vi "Username Dialog.vi"(7 "Address":string, 8 "Error In":errorcluster, 11 "Username In":string="cfield") -> (0 "Error Out":errorcluster, 3 "Username Out":string="cfield")   [LabVIEW 2017, in "Tests.lvlib"]
uses:
  Tests.lvlib
  <vilib>/Utility/miscctls.llb/LVSelectionTypeDef.ctl
panel:
  out "Host":string="USERNAME FOR TEST SERVER"
  in  "Cancel":bool
  in  "OK":bool
  in  "Username":string
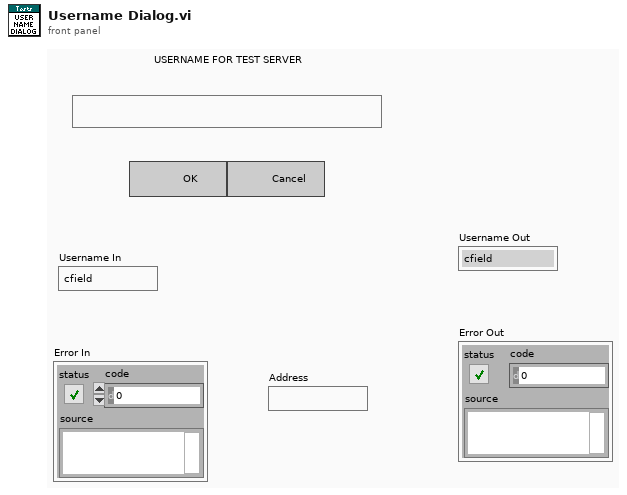
[diagram p1: front panel]
types:
  T1 = typedef "LVSelectionTypeDef.ctl" = cluster{"Selection Start":u32, "Selection End":u32}
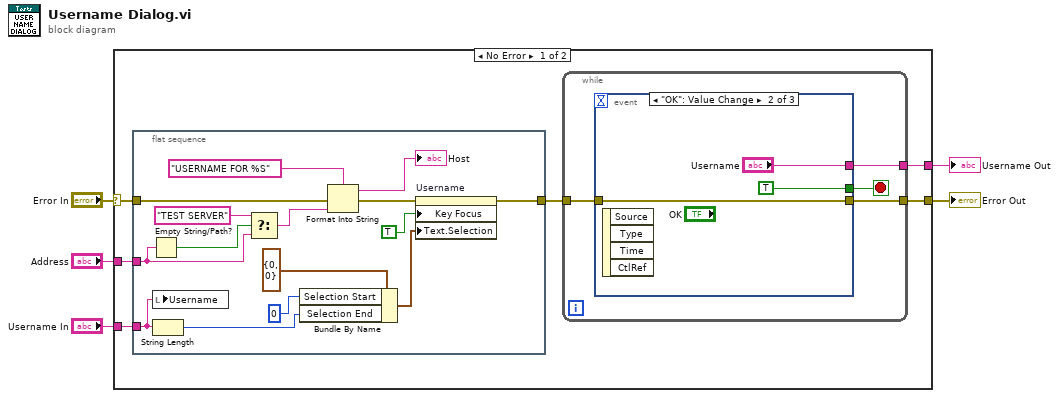
[diagram p0: block diagram]
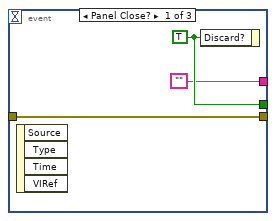
[diagram p2: hidden frame]
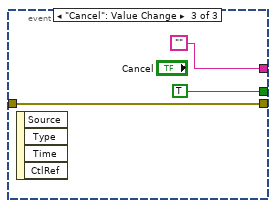
[diagram p3: hidden frame]
diagram:
  n1 = case shown="No Error" "Error In" {
    selector: "Error In" -> [w9 w40]
    tunnel: [w11 w40] -> w4
    tunnel: [w7 _] -> w3
    tunnel: "Username In" -> [w10 _]
    tunnel: "Address" -> [w6 _]
    frame No Error {
      n2 = flat-sequence {
        tunnel: w10 -> [w21]
        tunnel: w9 -> [w17]
        tunnel: [w26] -> w8
        tunnel: w6 -> [w14]
        frame #0 {
          n3 = Empty String/Path?(string/path=w14) -> (empty?=w19:bool)
          n4 = local write "Username"(w21) -> ()
          n5 = String Length(string=w21) -> (length=w20:i32)
          n6 = Select(t="TEST SERVER", s=w19, f=w14) -> (s? t:f=w12:string)
          n7 = Bundle By Name(cluster=T1 {"Selection Start"=0, "Selection End"=0} ("Text.Selection"), "Selection Start"=u32 0, "Selection End"=w20) -> (w23:T1)
          n8 = Format Into String(format string="USERNAME FOR %S", error in=w17, w12) -> (resulting string=→"Host":string, error out=w16:errorcluster)  [unwired: 1 in]
          n9 = property on="Username" class="Str"(error in=w16, "Key Focus"=TRUE, "Text.Selection"=w23) -> (error out=w26:errorcluster)  [unwired: 1 in, 1 out]
        }
      }
      n10 = while {
        tunnel: w8 -> [w29]
        tunnel: [w28] -> w11
        tunnel: [w27] -> w7
        stop <- w30 stop-if-true
        n11 = event shown="[1] \"OK\": Value Change" {
          selector: _ -> [_ _ _]
          dyn-events: _ -> [_ _ _]
          timeout: _ -> [_ _ _]
          tunnel: [w33 TRUE TRUE] -> w30
          tunnel: w29 -> [w32 w36 w39]
          tunnel: [w32 w36 w39] -> w28
          tunnel: ["" "Username" ""] -> w27
          event Panel Close? {
            w33 = TRUE
            n12 = event-data() -> ()  [unwired: 1 in, 4 out]
            n13 = event-data("Discard?"=w33) -> ()  [unwired: 1 in, 1 out]
          }
          event "OK": Value Change {
            n14 = event-data() -> ()  [unwired: 1 in, 4 out]
          }
          event "Cancel": Value Change {
            n15 = event-data() -> ()  [unwired: 1 in, 4 out]
          }
        }
      }
    }
    frame Error {
    }
  }
  "Error Out" <- w4
  "Username Out" <- w3
